vi "initialize eip tag lists.vi"(4 "output dictionary":refnum<class "data dictionary.lvclass">, 6 "input dictionary":refnum<class "data dictionary.lvclass">, 8 "error in":errorcluster, 10 "EthernetIP configuration in":refnum<class "EIP Tags Configuration.lvclass">, 11 "EthernetIP runtime in":refnum<class "EIP Tags Runtime.lvclass">) -> (0 "error out":errorcluster, 3 "EthernetIP runtime out":refnum<class "EIP Tags Runtime.lvclass">)   [LabVIEW 2013, in "EIP Tags Runtime.lvclass"]
uses:
  EIP Tags Runtime.lvclass
  configuration/EIP Tags Configuration.lvclass
  <vilib>/NI/Tag Bus/dictionary/data dictionary.lvclass
  <vilib>/ethernetip/ethernetip.llb/ethernetip.ctl
  configuration/EIP Tags Configuration.lvclass/EIP Tags Configuration.ctl
  eip tag spec.ctl
  configuration/eip tag types.ctl
  channel/EIP Tags Channel.lvclass/EIP Tags Channel.ctl
  <vilib>/NI/Tag Bus Module Framework/channel/TBM channel.lvclass/TBM channel.ctl
  <vilib>/NI/Tag Bus/tag/tag descriptor.lvclass/tag descriptor.ctl
  <vilib>/NI/Tag Bus/tag/Data Type.ctl
  EIP Tags Runtime.lvclass/EIP Tags Runtime.ctl
  channel/Read EIP Tag UUID.vi
  <vilib>/NI/Tag Bus Module Framework/channel/Read channel classification.vi
  <vilib>/NI/Tag Bus/tag/read tag name.vi
  <vilib>/NI/Tag Bus/tag/read data type.vi
  channel/Read element.vi
  configuration/Read Timeout (ms).vi
  configuration/Read EIP tags.vi
  configuration/read eip channels.vi
  <vilib>/ethernetip/ethernetip.llb/EthernetIP Tag Read Raw.vi
  channel/EIP Tags Channel.lvclass
  <vilib>/ethernetip/ethernetip.lvlib
  <vilib>/NI/Tag Bus/tag/tag descriptor.lvclass
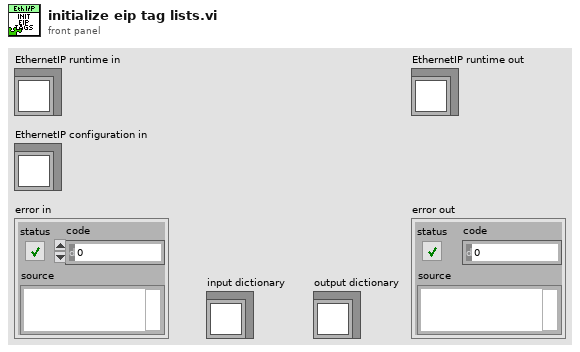
[diagram p1: front panel]
types:
  T1 = typedef "ethernetip.lvlib/ethernetip.ctl" = refnum<k21>
  T2 = typedef "EIP Tags Configuration.lvclass/eip tag definition.ctl" = cluster{"eip tag types":T3, "unique tag name":string, "Number of Elements":u32}
  T3 = typedef "EIP Tags Configuration.lvclass/eip tag types.ctl" = enum16{"SINT", "INT", "DINT", "REAL", "BOOL", "STRING"}
  T4 = typedef "EIP Tags Runtime.lvclass/eip tag spec.ctl" = cluster{"eip tag types":T3, "Network Path":string, "Tag Name":string, "Number of Elements":u32, "data indices":i32[], "tag bus indices":i32[], "array tbtag":bool}
  T5 = typedef "tag bus.lvlib/tag descriptor.lvclass/Data Type.ctl" = enum16{"Double", "Single", "I64", "I32", "I16", "I8", "U64", "U32", "U16", "U8", "Boolean", "String", "Array of Double", "Array of Single", "Array of I64", "Array of I32", "Array of I16", "Array of I8", "Array of U64", "Array of U32", "Array of U16", "Array of U8", "Array of Boolean", "Array of String"}
  T6 = typedef "TBM channel.lvclass/channel classification.ctl" = enum16{"input data", "output data", "processing parameter", "processing result"}
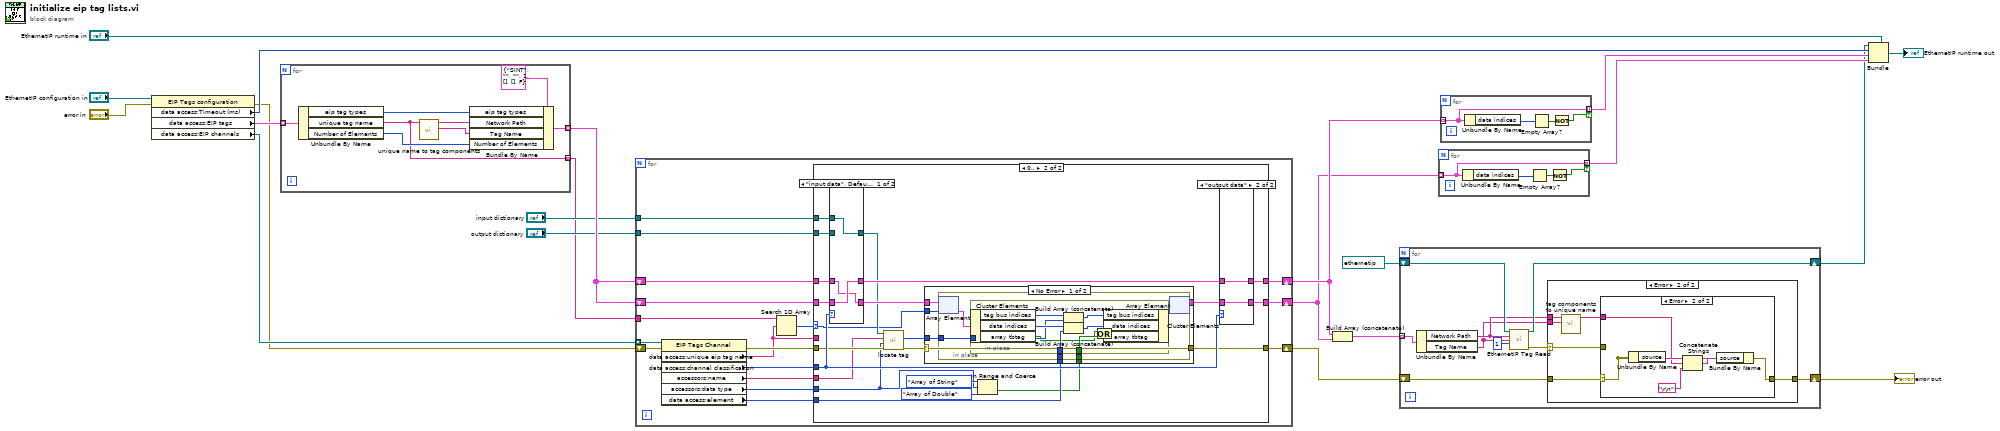
[diagram p0: block diagram]
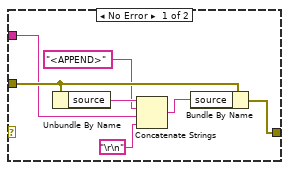
[diagram p3: hidden frame]
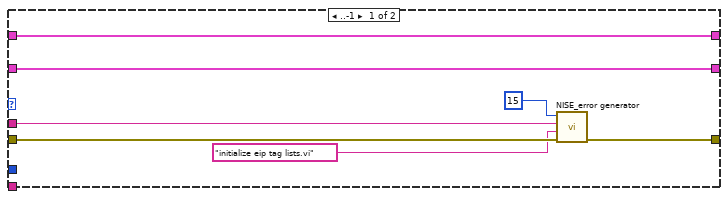
[diagram p4: hidden frame]
diagram:
  n1 = property class="EIP Tags configuration"(reference="EthernetIP configuration in", error in="error in") -> (error out=w11:errorcluster, "data access:Timeout (ms)"=w17:i32, "data access:EIP tags"=w16:T2[], "data access:EIP channels"=w14:refnum<class "EIP Tags Channel.lvclass">[])  [unwired: 1 out]
  n2 = for {
    tunnel: w16 -> [w29] mode=indexing
    tunnel: [w23] -> w15 mode=indexing
    tunnel: [w22] -> w8 mode=indexing
    n3 = Unbundle By Name(w29) -> ("eip tag types"=w27:T3, "unique tag name"=w22:string, "Number of Elements"=w26:u32)
    n4 = call "unique name to tag components.vi"("unique name"=w22) -> ("Tag Name"=w24:string, "Network Path"=w25:string)  [unwired: 9 in]
    n5 = Bundle By Name(cluster=T4 {"eip tag types"=enum."SINT", "Network Path"="", "Tag Name"="", "Number of Elements"=1, "data indices"=[], "tag bus indices"=[], "array tbtag"=FALSE} ("tag spec"), "eip tag types"=w27, "Network Path"=w25, "Tag Name"=w24, "Number of Elements"=w26) -> (w23:T4)
  }
  n6 = for {
    shift-right: [w41] -> w5
    shift-left: w15 -> [w42]
    shift-right: [w39] -> w4
    shift-left: w15 -> [w40]
    tunnel: w14 -> [w45] mode=indexing
    tunnel: "input dictionary" -> [w36]
    tunnel: "output dictionary" -> [w35]
    shift-right: [w37] -> w2
    shift-left: w11 -> [w46]
    tunnel: w8 -> [w44]
    n7 = property class="EIP Tags Channel"(reference=w45, error in=w46) -> (error out=w38:errorcluster, "data access:unique eip tag name"=w34:string, "data access:channel classification"=w33:T6, "accessors:name"=w31:string, "accessors:data type"=w30:T5, "data access:element"=w32:i32)  [unwired: 1 out]
    n8 = Search 1D Array(1D array=w44, element=w34) -> (index of element=w43:i32)  [unwired: 1 in]
    n9 = case shown="0.." w43 {
      selector: w43 -> [_ w60]
      tunnel: w42 -> [w53 w73]
      tunnel: [w53 w71] -> w41
      tunnel: w40 -> [w52 w72]
      tunnel: [w52 w70] -> w39
      tunnel: w38 -> [w51 w65]
      tunnel: [w50 w61] -> w37
      tunnel: w36 -> [_ w74]
      tunnel: w35 -> [_ w75]
      tunnel: w34 -> [w48 _]
      tunnel: w33 -> [_ w68]
      tunnel: w32 -> [_ w58]
      tunnel: w31 -> [_ w63]
      tunnel: w30 -> [_ w55]
      frame ..-1 {
        n10 = call <vilib>:"NISE_error generator.vi"("error in"=w51, "source"="initialize eip tag lists.vi", "append error message"=w48, "error code (0)"=15) -> ("error out"=w50:errorcluster)  [unwired: 5 in]
      }
      frame 0.. {
        n11 = case shown="\"input data\", Default" w68 {
          tunnel: [w105 w108] -> w64
          tunnel: w75 -> [_ w108]
          tunnel: w74 -> [w105 _]
          tunnel: w73 -> [w103 w106]
          tunnel: w72 -> [w104 w107]
          tunnel: [w103 w107] -> w67
          tunnel: [w104 w106] -> w69
          frame "input data", Default {
          }
          frame "output data" {
          }
        }
        n12 = call <vilib>:"locate tag.vi"("error in"=w65, "data type"=w55, "name"=w63, "data dictionary in"=w64) -> ("error out"=w62:errorcluster, "index"=w59:i32)  [unwired: 5 in, 1 out]
        n13 = In Range and Coerce(upper limit=Data_Type."Array of String", x=w55, lower limit=Data_Type."Array of Double") -> (In Range?=w54:bool)  [unwired: 1 out]
        n14 = case shown="No Error" w62 {
          selector: w62 -> [w80 w98]
          tunnel: w67 -> [w82 w97]
          tunnel: [w81 w97] -> w66
          tunnel: [w80 w98] -> w61
          tunnel: w60 -> [w79 _]
          tunnel: w59 -> [w78 _]
          tunnel: w58 -> [w77 _]
          tunnel: w54 -> [w76 _]
          frame No Error {
            n15 = in-place {
              in-place-border: w78 -> [w85]
              in-place-border: w77 -> [w84]
              in-place-border: w76 -> [w83]
              n16 = in-place-array #1(w82, w79) -> (w87:T4)
              n17 = in-place {
                in-place-border: w85 -> [w92]
                in-place-border: w84 -> [w91]
                in-place-border: w83 -> [w90]
                n18 = in-place-cluster #2(w87) -> ("tag bus indices"=w95:i32[], "data indices"=w96:i32[], "array tbtag"=w88:bool)
                n19 = Build Array (concatenate)(w95, w92) -> (w94:i32[])
                n20 = Build Array (concatenate)(w96, w91) -> (w93:i32[])
                n21 = Or(x=w88, y=w90) -> (x .or. y?=w89:bool)
                n22 = in-place-cluster #2("tag bus indices"=w94, "data indices"=w93, "array tbtag"=w89) -> (w86:T4)
              }
              n23 = in-place-array #1(w86) -> (w81:T4[])  [unwired: 1 out]
            }
          }
          frame Error {
          }
        }
        n24 = case shown="\"output data\"" w68 {
          tunnel: w69 -> [w99 w101]
          tunnel: w66 -> [w100 w102]
          tunnel: [w99 w102] -> w70
          tunnel: [w100 w101] -> w71
          frame "input data", Default {
          }
          frame "output data" {
          }
        }
      }
    }
  }
  n25 = Build Array (concatenate)(w5, w4) -> (w3:T4[])
  n26 = for {
    shift-right: [w116] -> w6
    shift-left: T1 "Default" ("Session in") -> [w117]
    tunnel: w3 -> [w115] mode=indexing
    shift-right: [w112] -> w1
    shift-left: w2 -> [w111]
    n27 = Unbundle By Name(w115) -> ("Network Path"=w110:string, "Tag Name"=w109:string)
    n28 = call-poly <vilib>:"EthernetIP Tag Read.vi"("Session in"=w117, "Network Path"=w110, "Tag Name"=w109, "Number of Elements"=u32 1) -> ("Session out"=w116:T1, "error out"=w113:errorcluster)  [unwired: 9 in, 1 out]
    n29 = case shown="Error" w113 {
      selector: w113 -> [_ w122]
      tunnel: [w118 w123] -> w112
      tunnel: w111 -> [w118 w124]
      tunnel: w110 -> [_ w121]
      tunnel: w109 -> [_ w120]
      frame No Error {
      }
      frame Error {
        n30 = call "tag components to unique name.vi"("Tag Name"=w120, "Network Path"=w121) -> ("unique name"=w119:string)  [unwired: 9 in]
        n31 = case shown="Error" w124 {
          selector: w124 -> [_ w132]
          tunnel: [w130 w137] -> w123
          tunnel: w122 -> [w131 _]
          tunnel: w119 -> [w125 w133]
          frame No Error {
            n32 = Unbundle By Name(w131) -> ("source"=w128:string)
            n33 = Concatenate Strings(w128, "<APPEND>" ("string"), w125, "\r\n") -> (w129:string)
            n34 = Bundle By Name(cluster=w131, "source"=w129) -> (w130:errorcluster)
          }
          frame Error {
            n35 = Unbundle By Name(w132) -> ("source"=w135:string)
            n36 = Concatenate Strings(w135, w133, "\r\n") -> (w136:string)
            n37 = Bundle By Name(cluster=w132, "source"=w136) -> (w137:errorcluster)
          }
        }
      }
    }
  }
  "error out" <- w1
  n38 = for {
    tunnel: w4 -> [w139] mode=indexing
    tunnel: [w139] -> w9 mode=indexing if=w138
    n39 = Unbundle By Name(w139) -> ("data indices"=w141:i32[])
    n40 = Empty Array?(array=w141) -> (empty?=w140:bool)
    n41 = Not(x=w140) -> (.not. x?=w138:bool)
  }
  n42 = for {
    tunnel: w5 -> [w143] mode=indexing
    tunnel: [w143] -> w10 mode=indexing if=w142
    n43 = Unbundle By Name(w143) -> ("data indices"=w145:i32[])
    n44 = Empty Array?(array=w145) -> (empty?=w144:bool)
    n45 = Not(x=w144) -> (.not. x?=w142:bool)
  }
  n46 = Bundle(cluster="EthernetIP runtime in", w6, w17, w10, w9) -> (→"EthernetIP runtime out":refnum<class "EIP Tags Runtime.lvclass">)
